vi "Common Device Queue Get Command.vi"(0 "Common Queue":refnum<queue>, 11 "Notifier Name":string) -> (4 "Common Queue":refnum<queue>, 8 "Command":string)   [LabVIEW 2016]
panel:
  out "Queue Element":string
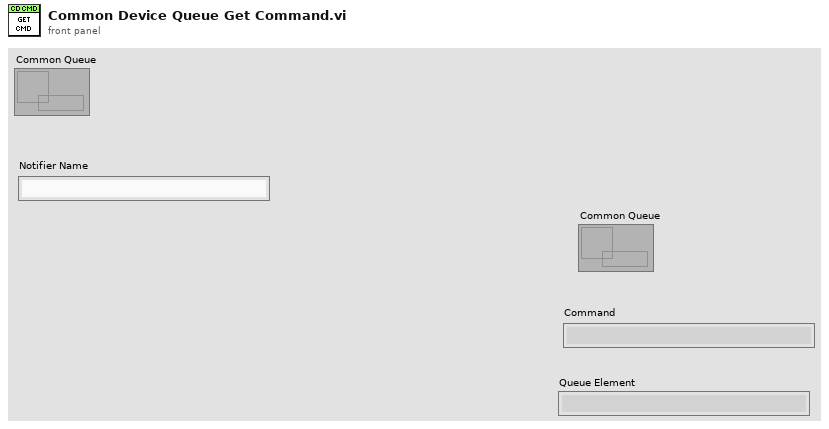
[diagram p1: front panel]
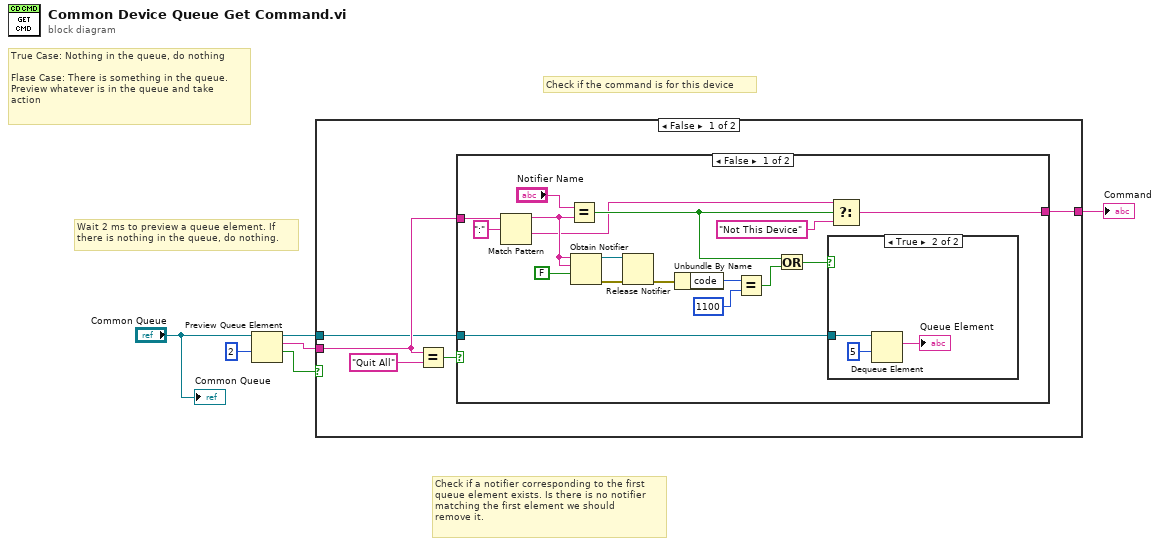
[diagram p0: block diagram]
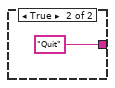
[diagram p3: hidden frame]
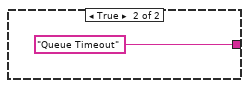
[diagram p4: hidden frame]
diagram:
  # "True Case: Nothing in the queue, do nothing\n\nFlase Case: There is something in the queue.\nPreview whatever is in the queue and take\naction"
  # "Wait 2 ms to preview a queue element. If\nthere is nothing in the queue, do nothing."
  # "Check if a notifier corresponding to the first\nqueue element exists. Is there is no notifier\nmatching the first element we should\nremove it."
  # "Check if the command is for this device"
  n1 = Preview Queue Element(queue="Common Queue", timeout in ms (-1)=2) -> (queue out=w4:refnum<queue>, element=w5:string, timed out?=w1:bool)  [unwired: 1 in, 1 out]
  n2 = case shown="False" w1 {
    tunnel: [w11 "Queue Timeout" ("t")] -> w6
    tunnel: w5 -> [w8 _]
    tunnel: w4 -> [w7 _]
    frame False {
      n3 = Equal?(x=w8, y="Quit All" ("regular expression")) -> (x = y?=w9:bool)
      n4 = case shown="False" w9 {
        tunnel: w7 -> [w18 _]
        tunnel: [w17 "Quit" ("t")] -> w11
        tunnel: w8 -> [w16 _]
        frame False {
          n5 = Match Pattern(string=w16, regular expression=":") -> (before substring=w24:string, after substring=w23:string)  [unwired: 1 in, 2 out]
          n6 = Equal?(x="Notifier Name", y=w24) -> (x = y?=w26:bool)
          n7 = Obtain Notifier(name (unnamed)=w24, notification data type=w24, create if not found? (T)=FALSE) -> (notifier out=w15:refnum<notifier>, error out=w14:errorcluster)  [unwired: 1 in, 1 out]
          n8 = Release Notifier(notifier=w15, error in (no error)=w14) -> (error out=w13:errorcluster)  [unwired: 1 in, 2 out]
          n9 = Unbundle By Name(w13) -> ("code"=w25:i32)
          n10 = Equal?(x=w25, y=1100) -> (x = y?=w27:bool)
          n11 = Or(x=w26, y=w27) -> (x .or. y?=w28:bool)
          n12 = case shown="True" w28 {
            tunnel: w18 -> [_ w29]
            frame False {
            }
            frame True {
              n13 = Dequeue Element(queue=w29, timeout in ms (-1)=5) -> (element=→"Queue Element":string)  [unwired: 1 in, 3 out]
            }
          }
          n14 = Select(t=w23, s=w26, f="Not This Device") -> (s? t:f=w17:string)
        }
        frame True {
        }
      }
    }
    frame True {
    }
  }
  "Command" <- w6
  "Common Queue" <- "Common Queue"
